vi "BaseProvider_GetStaticMethods.vi"(1 "ClassTemplateName":string, 3 "ConnectorPaneSettings":string, 5 "error in":errorcluster) -> (15 "NormalMethods":T1[](array[typedef]), 19 "error out":errorcluster)   [LabVIEW 2020]
uses:
  Provider_LvNativeClass/ClassWriterNative_class/MethodInfo.ctl
  Provider_LvNativeClass/ClassWriterNative_class/MethodType.ctl
  Provider_LvNativeClass/ClassWriterNative_class/MethodInfo_Option.ctl
  <vilib>/Utility/config.llb/Read Key (String).vi
  <vilib>/Utility/config.llb/NI_LVConfig.lvlib
  Provider_LvNativeClass/ClassWriterNative_class/ClassWriterNative.lvclass
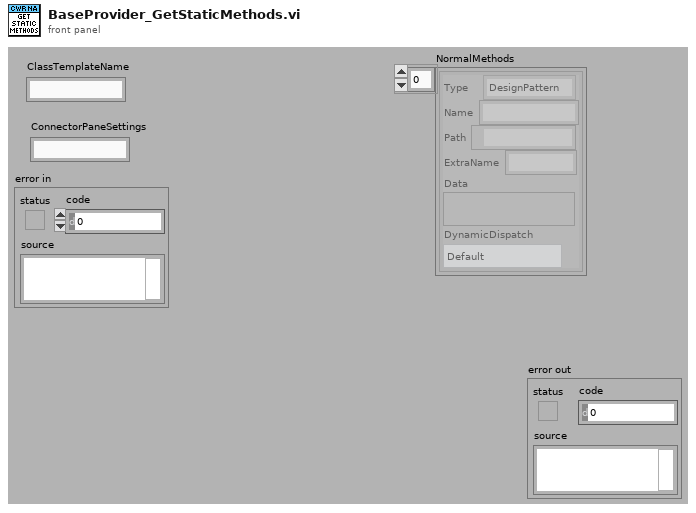
[diagram p1: front panel]
types:
  T1 = typedef "ClassWriterNative.lvclass/MethodInfo.ctl" = cluster{"Type":T2, "Name":string, "Path":path, "ExtraName":string, "Data":variant, "DynamicDispatch":T3}
  T2 = typedef "ClassWriterNative.lvclass/MethodType.ctl" = enum16{"Normal", "MethodPlugIn", "DesignPattern", "AF-Method"}
  T3 = typedef "ClassWriterNative.lvclass/MethodInfo_Option.ctl" = enum16{"Default", "OnAtStart", "OffAtStart", "AlwaysOn", "AlwaysOff"}
  T4 = typedef "NI_LVConfig.lvlib/Config Data RefNum.ctl" = refnum<k1>
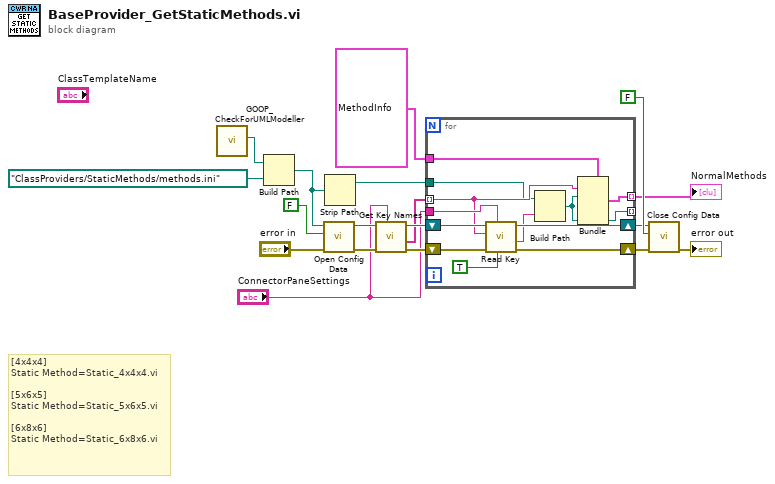
[diagram p0: block diagram]
diagram:
  # "[4x4x4]\nStatic Method=Static_4x4x4.vi\n\n[5x6x5]\nStatic Method=Static_5x6x5.vi\n\n[6x8x6]\nStatic Method=Static_6x8x6.vi"
  n1 = call "GOOP_CheckForUMLModeller.vi"() -> ("UML-Modeller VI Path"=w1:path)  [unwired: 10 in, 1 out]
  n2 = Build Path(base path=w1, name or relative path=path "ClassProviders/StaticMethods/methods.ini" ("base path")) -> (appended path=w4:path)
  n3 = call <vilib>:"Open Config Data.vi"("error in (no error)"="error in", "create file if necessary (T)"=FALSE ("create file if necessary? (T)"), "configuration file path"=w4) -> ("error out"=w10:errorcluster, "refnum"=w9:T4)  [unwired: 6 in, 1 out]
  n4 = Strip Path(path=w4) -> (stripped path=w3:path)  [unwired: 1 out]
  n5 = call <vilib>:"Get Key Names.vi"("section"="ConnectorPaneSettings", "error in (no error)"=w10, "refnum"=w9) -> ("error out"=w8:errorcluster, "key names"=w6:string[], "refnum out"=w7:T4)  [unwired: 5 in, 1 out]
  n6 = for {
    shift-right: [w26] -> w12
    shift-left: w8 -> [w29]
    shift-right: [w27] -> w13
    shift-left: w7 -> [w30]
    tunnel: "ConnectorPaneSettings" -> [w28]
    tunnel: w6 -> [w22] mode=indexing
    tunnel: [w24] -> w2 mode=indexing
    tunnel: T1 {"Type"=enum."Normal", "Name"="", "Path"=path "", "ExtraName"="", "Data"=variant, "DynamicDispatch"=enum."Default"} ("Cluster") -> [w25]
    tunnel: [w19] -> _ mode=indexing
    tunnel: w3 -> [w21]
    n7 = call-poly <vilib>:"Read Key.vi"("read raw string? (F)"=TRUE, "section"=w28, "error in (no error)"=w29, "key"=w22, "refnum"=w30) -> ("error out"=w26:errorcluster, "value"=w20:string, "refnum out"=w27:T4)  [unwired: 3 in, 1 out]
    n8 = Build Path(base path=w21, name or relative path=w20) -> (appended path=w19:path)
    n9 = Bundle(cluster=w25, "Name"=w22, "Path"=w19) -> (w24:T1)  [unwired: 4 in]
  }
  "NormalMethods" <- w2
  n10 = call <vilib>:"Close Config Data.vi"("error in (no error)"=w12, "write file if changed (T)"=FALSE ("create file if necessary? (T)"), "refnum"=w13) -> ("error out"=→"error out":errorcluster)  [unwired: 7 in, 1 out]
